vi "Camera_Grab.vi"(8 "error in (no error)":errorcluster, 11 "TCP Network Connection in":refnum<k5>) -> (0 "error out":errorcluster, 1 "Image":u8[][](array[numeric]), 2 "Length":u32, 3 "TCP Network Connection out":refnum<k5>, 4 "Part ID":u32, 5 "Status":u8)   [LabVIEW 2018]
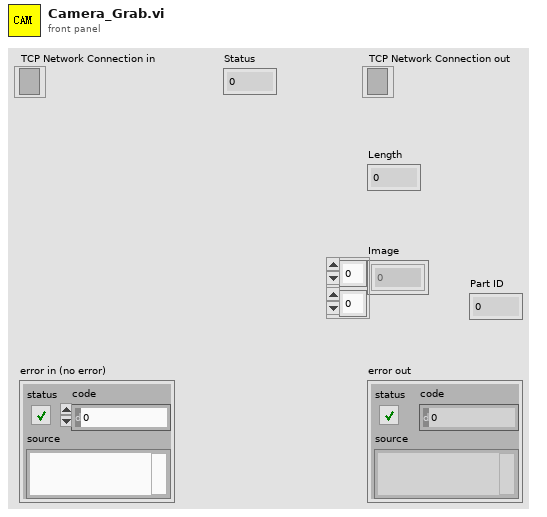
[diagram p1: front panel]
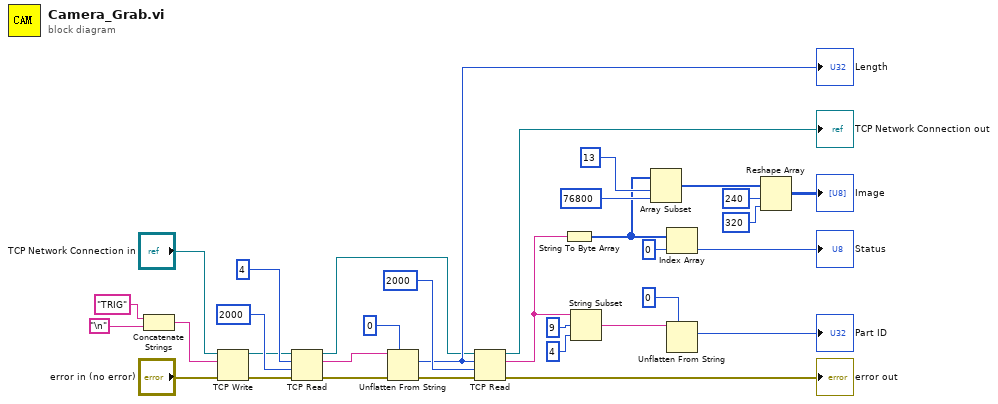
[diagram p0: block diagram]
diagram:
  n1 = Concatenate Strings("TRIG" ("address"), "\n") -> (w9:string)
  n2 = TCP Write(connection ID="TCP Network Connection in", data in=w9, error in (no error)="error in (no error)") -> (connection ID out=w12:refnum<k5>, error out=w13:errorcluster)  [unwired: 1 in, 1 out]
  n3 = TCP Read(connection ID=w12, bytes to read=4, error in (no error)=w13, 9:2000 ("timeout ms (25000)")) -> (connection ID out=w19:refnum<k5>, data out=w16:string, error out=w18:errorcluster)  [unwired: 1 in]
  n4 = Unflatten From String(type=u32 0 ("bytes to read"), binary string=w16, error in (no error)=w18) -> (value=w21:u32, error out=w20:errorcluster)  [unwired: 2 in, 1 out]
  "Length" <- w21
  n5 = TCP Read(connection ID=w19, bytes to read=w21, error in (no error)=w20, 9:2000 ("timeout ms (25000)")) -> (connection ID out=→"TCP Network Connection out":refnum<k5>, data out=w6:string, error out=→"error out":errorcluster)  [unwired: 1 in]
  n6 = String To Byte Array(string=w6) -> (unsigned byte array=w25:u8[])
  n7 = String Subset(string=w6, offset (0)=9, length (rest)=4 ("length (rest)")) -> (substring=w3:string)
  n8 = Array Subset(array=w25, index=13, length=76800) -> (w28:u8[])
  n9 = Index Array(array=w25, index=0) -> (element=→"Status":u8)
  n10 = Unflatten From String(type=u32 0, binary string=w3) -> (value=→"Part ID":u32)  [unwired: 3 in, 2 out]
  n11 = Reshape Array(w28, 240 ("dimension size"), 320 ("dimension size")) -> (→"Image":u8[][])
